vi "Start Test.vi"(8 "error in (no error)":errorcluster, 10 "Tests":string[](array[string]), 11 "Result Model by Reference In":refnum<class "Result Model.lvclass">) -> (0 "error out":errorcluster)   [LabVIEW 2020, in "Result Model.lvclass"]
uses:
  Result Model/Result Model.lvclass
  Result Model/Result Model.lvclass/Result Model.ctl
  Core/Result/Status.ctl
  6371cb2c-8366-4971-afb8-488d017e4980.vi
  Core/Result/Result.lvlib
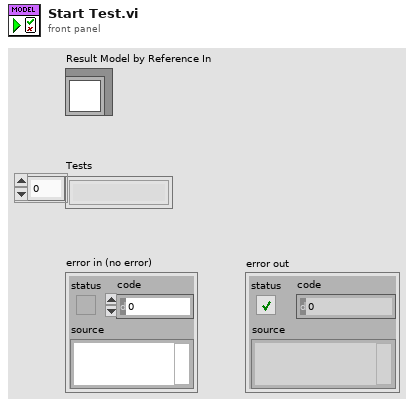
[diagram p1: front panel]
types:
  T1 = typedef "Result.lvlib/Status.ctl" = enum16{"", "Passed", "Failed", "Error", "Skipped", "Setup Error", "Broken", "Teardown Error"}
  T2 = typedef "Result.lvlib/Type.ctl" = enum16{"Test Case", "Test Suite", "Test Run", "Pass", "Fail", "Skip", "Pass if", "Fail if", "Pass if Error", "Fail if Error", "Pass if Equal", "Fail if Equal"}
  T3 = cluster{"Tests":string[], "Run Queue":string[], "Test Statuses":map{string, T1}, "Execution Time":map{string, dbl}, "Assertions":map{string, cluster{"Result Type":T2, "Status":T1, "Description":string, "Data":cluster{"Expected":variant, "Actual":variant, "Delta":variant}}[]}}
  T4 = map{string, cluster{"Result Type":T2, "Status":T1, "Description":string, "Data":cluster{"Expected":variant, "Actual":variant, "Delta":variant}}[]}
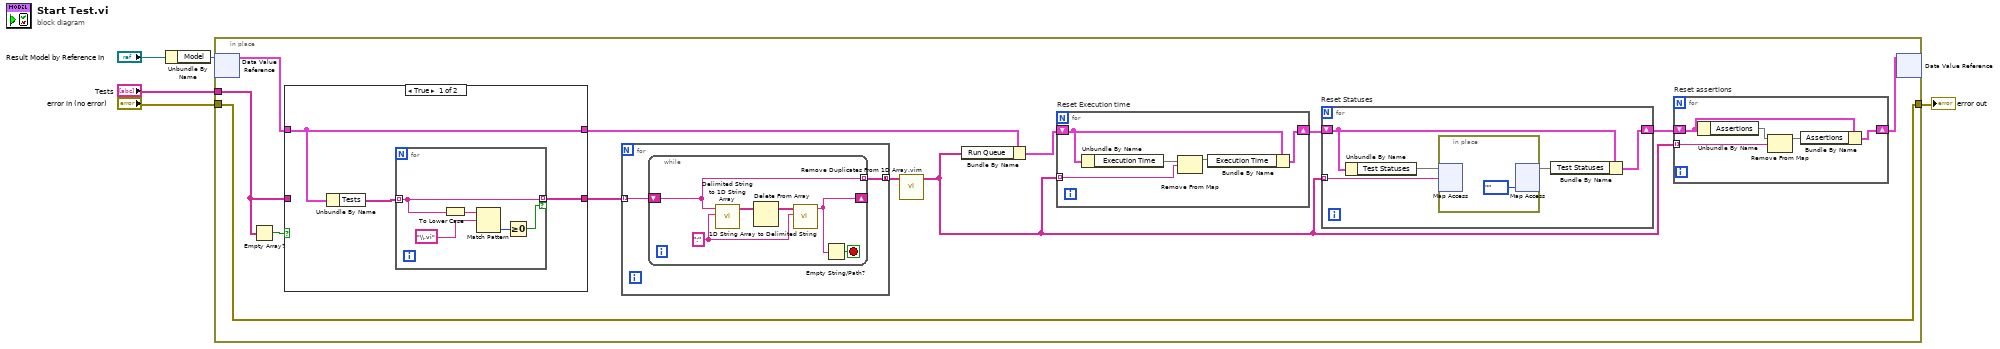
[diagram p0: block diagram]
diagram:
  n1 = Unbundle By Name("Result Model by Reference In") -> ("Model"=w4:refnum<data-value>)
  n2 = in-place {
    in-place-border: "error in (no error)" -> [w6]
    in-place-border: [w6] -> w2
    in-place-border: "Tests" -> [w15]
    n3 = in-place-dvr #1(w4) -> (w16:T3)  [unwired: 1 out]
    n4 = Empty Array?(array=w15) -> (empty?=w7:bool)
    n5 = case shown="True" w7 {
      tunnel: w16 -> [w19 w27]
      tunnel: [w19 w27] -> w9
      tunnel: w15 -> [_ w26]
      tunnel: [w18 w26] -> w8
      frame True {
        n6 = Unbundle By Name(w19) -> ("Tests"=w20:string[])
        n7 = for {
          tunnel: w20 -> [w25] mode=indexing
          tunnel: [w25] -> w18 mode=indexing if=w21
          n8 = To Lower Case(string=w25) -> (all lower case string=w22:string)
          n9 = Match Pattern(string=w22, regular expression="\\.vi") -> (offset past match=w23:i32)  [unwired: 1 in, 3 out]
          n10 = Greater Or Equal To 0?(x=w23) -> (x >= 0?=w21:bool)
        }
      }
      frame False {
      }
    }
    n11 = for {
      tunnel: w8 -> [w29] mode=indexing
      tunnel: [w28] -> w13 mode=concatenating
      n12 = while {
        shift-right: [w31] -> _
        shift-left: w29 -> [w30]
        tunnel: [w30] -> w28 mode=indexing
        stop <- w32 stop-if-true
        w34 = ":" ("delimiter")
        n13 = call <vilib>:"Delimited String to 1D String Array.vi"("delimiter"=w34, "delimited string"=w30) -> ("string array"=w35:string[])  [unwired: 9 in]
        n14 = Delete From Array(array=w35) -> (array with subset deleted=w33:string[])  [unwired: 2 in, 1 out]
        n15 = call <vilib>:"1D String Array to Delimited String.vi"("delimiter"=w34, "string array"=w33) -> ("delimited string"=w31:string)  [unwired: 9 in]
        n16 = Empty String/Path?(string/path=w31) -> (empty?=w32:bool)
      }
    }
    n17 = call "Remove Duplicates From 1D Array.vim"("array"=w13) -> ("array with duplicates removed"=w14:string[])  [unwired: 10 in]
    n18 = Bundle By Name(cluster=w9, "Run Queue"=w14) -> (w12:T3)
    n19 = for "Reset Execution time" {
      tunnel: w14 -> [w40] mode=indexing
      shift-right: [w36] -> w11
      shift-left: w12 -> [w37]
      n20 = Unbundle By Name(w37) -> ("Execution Time"=w39:map{string, dbl})
      n21 = Remove From Map(10:w40, 11:w39) -> (3:w38:map{string, dbl})  [unwired: 2 out]
      n22 = Bundle By Name(cluster=w37, "Execution Time"=w38) -> (w36:T3)
    }
    n23 = for "Reset Statuses" {
      tunnel: w14 -> [w45] mode=indexing
      shift-right: [w41] -> w10
      shift-left: w11 -> [w42]
      n24 = Unbundle By Name(w42) -> ("Test Statuses"=w44:map{string, T1})
      n25 = in-place {
        n26 = in-place-map #2(w44, w45) -> ()  [unwired: 1 in, 2 out]
        n27 = in-place-map #2(Status."" ("value")) -> (w43:map{string, T1})  [unwired: 1 in, 2 out]
      }
      n28 = Bundle By Name(cluster=w42, "Test Statuses"=w43) -> (w41:T3)
    }
    n29 = for "Reset assertions" {
      tunnel: w14 -> [w51] mode=indexing
      shift-right: [w47] -> w17
      shift-left: w10 -> [w48]
      n30 = Unbundle By Name(w48) -> ("Assertions"=w50:T4)
      n31 = Remove From Map(10:w51, 11:w50) -> (3:w49:T4)  [unwired: 2 out]
      n32 = Bundle By Name(cluster=w48, "Assertions"=w49) -> (w47:T3)
    }
    n33 = in-place-dvr #1(w17) -> ()  [unwired: 2 out]
  }
  "error out" <- w2
